vi "Read TDMS File.vi"(11 "文件路径":path) -> (3 "数据系列":T1[](array[typedef]))   [LabVIEW 2020, in "Data Viewer.lvlib" / "Data Viewer.lvclass"]
uses:
  Data Viewer.lvclass
  Data Serie--cluster.ctl
  Data Viewer.lvlib
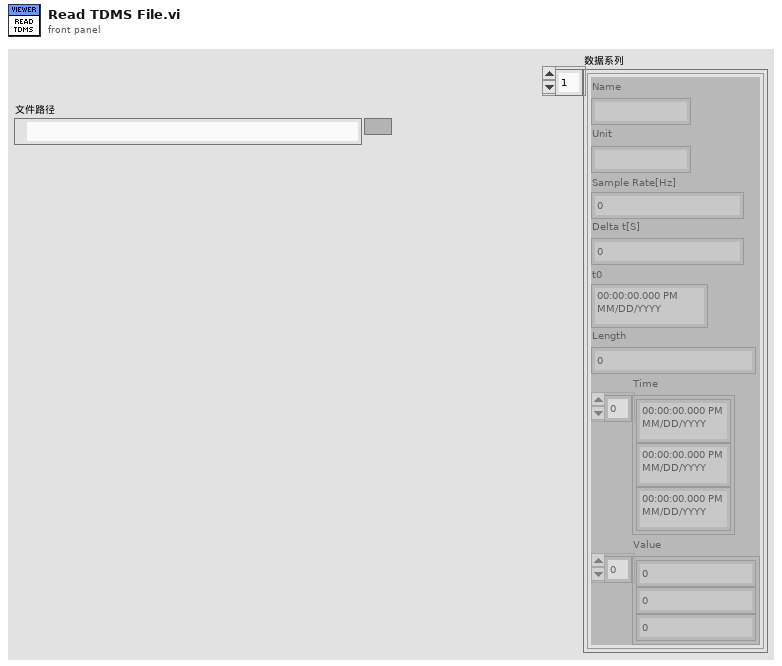
[diagram p1: front panel]
types:
  T1 = typedef "Data Viewer.lvlib/Data Serie--cluster.ctl" = cluster{"Name":string, "Unit":string, "Sample Rate[Hz]":dbl, "Delta t[S]":dbl, "t0":timestamp, "Length":i32, "Time":timestamp[], "Value":dbl[]}
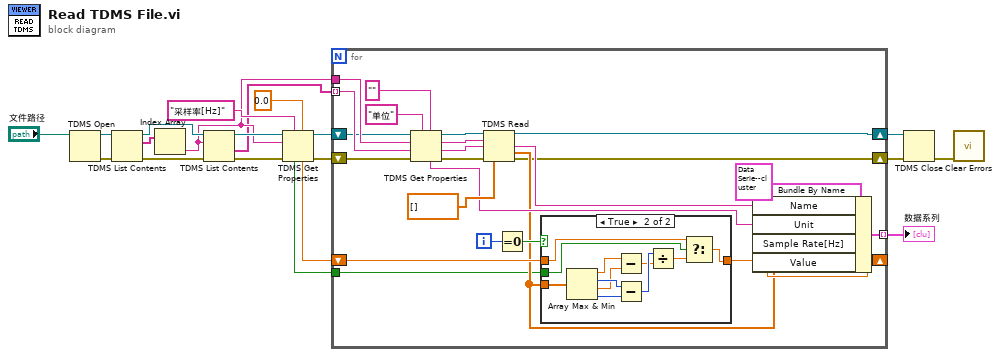
[diagram p0: block diagram]
diagram:
  n1 = TDMS Open(11:"文件路径") -> (0:w18:errorcluster, 3:w19:refnum<k34>)  [unwired: 6 in]
  n2 = TDMS List Contents(4:w18, 7:w19) -> (0:w12:errorcluster, 2:w15:string[], 3:w14:refnum<k34>)  [unwired: 1 in, 1 out]
  n3 = Index Array(array=w15) -> (element=w10:string)  [unwired: 1 in]
  n4 = TDMS List Contents(4:w12, 6:w10, 7:w14) -> (0:w11:errorcluster, 1:w9:string[], 3:w13:refnum<k34>)  [unwired: 1 out]
  n5 = TDMS Get Properties(5:0.0, 7:"采样率[Hz]" ("属性名称"), 8:w11, 10:w10, 11:w13) -> (0:w6:errorcluster, 3:w8:refnum<k34>, 4:w4:dbl, 6:w2:bool)  [unwired: 1 in, 2 out]
  n6 = for {
    tunnel: w10 -> [w43]
    tunnel: w9 -> [w42] mode=indexing
    shift-right: [w24] -> w7
    shift-left: w8 -> [w41]
    shift-right: [w25] -> w5
    shift-left: w6 -> [w40]
    shift-right: [w27] -> _
    shift-left: w4 -> [w28]
    tunnel: [w23] -> w3 mode=indexing
    tunnel: w2 -> [w22]
    i -> [w30]
    n7 = TDMS Get Properties(5:"", 7:"单位" ("属性名称"), 8:w40, 9:w42, 10:w43, 11:w41) -> (0:w36:errorcluster, 1:w34:string, 2:w35:string, 3:w37:refnum<k34>, 4:w31:string)  [unwired: 1 out]
    n8 = TDMS Read(0:w37, 5:w35, 7:w34, 11:w36, 12:dbl[] []) -> (4:w24:refnum<k34>, 8:w32:string, 10:w26:dbl[], 15:w25:errorcluster)  [unwired: 3 in, 2 out]
    n9 = Equal To 0?(x=w30) -> (x = 0?=w29:bool)
    n10 = case shown="True" w29 {
      tunnel: w28 -> [w44 w45]
      tunnel: [w44 w55] -> w27
      tunnel: w26 -> [_ w48]
      tunnel: w22 -> [_ w47]
      frame False {
      }
      frame True {
        n11 = Array Max & Min(array=w48) -> (max value=w50:dbl, max index (indices)=w52:i32, min value=w51:dbl, min index (indices)=w49:i32)
        n12 = Subtract(x=w50, y=w51) -> (x-y=w53:dbl)
        n13 = Subtract(x=w52, y=w49) -> (x-y=w54:i32)
        n14 = Divide(x=w54, y=w53) -> (x/y=w46:dbl)
        n15 = Select(t=w45, s=w47, f=w46) -> (s? t:f=w55:dbl)
      }
    }
    n16 = Bundle By Name(cluster=T1 {"Name"="", "Unit"="", "Sample Rate[Hz]"=0.0, "Delta t[S]"=0.0, "t0"=timestamp(0 s since 1904-01-01), "Length"=0, "Time"=[], "Value"=[]} ("Data Serie"), "Name"=w32, "Unit"=w31, "Sample Rate[Hz]"=w27, "Value"=w26) -> (w23:T1)
  }
  "数据系列" <- w3
  n17 = TDMS Close(8:w5, 11:w7) -> (0:w1:errorcluster)  [unwired: 1 out]
  n18 = call <vilib>:"Clear Errors.vi"("error in (no error)"=w1) -> ()  [unwired: 5 in, 2 out]
